vi "sinewave_recovery_array__1dabf32195.vi"(7 "stop steps":i32, 8 "# periods":dbl, 9 "recovery phase (32 points half period)":dbl, 10 "amplitude":dbl=1.0 format="%0.2p", 11 "frequency":dbl=10.0 format="%0.2p") -> (0 "expected duration":dbl, 1 "total points":i32, 2 "Waveform Graph":dbl[](graph), 3 "shear points":dbl)   [LabVIEW 2023]
uses:
  <vilib>/Analysis/NI_AALBase.lvlib
panel:
  out "element":dbl
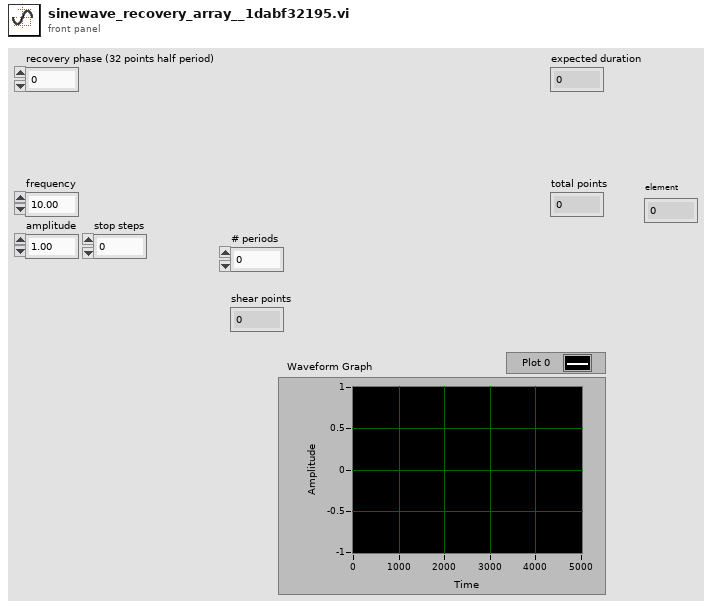
[diagram p1: front panel]
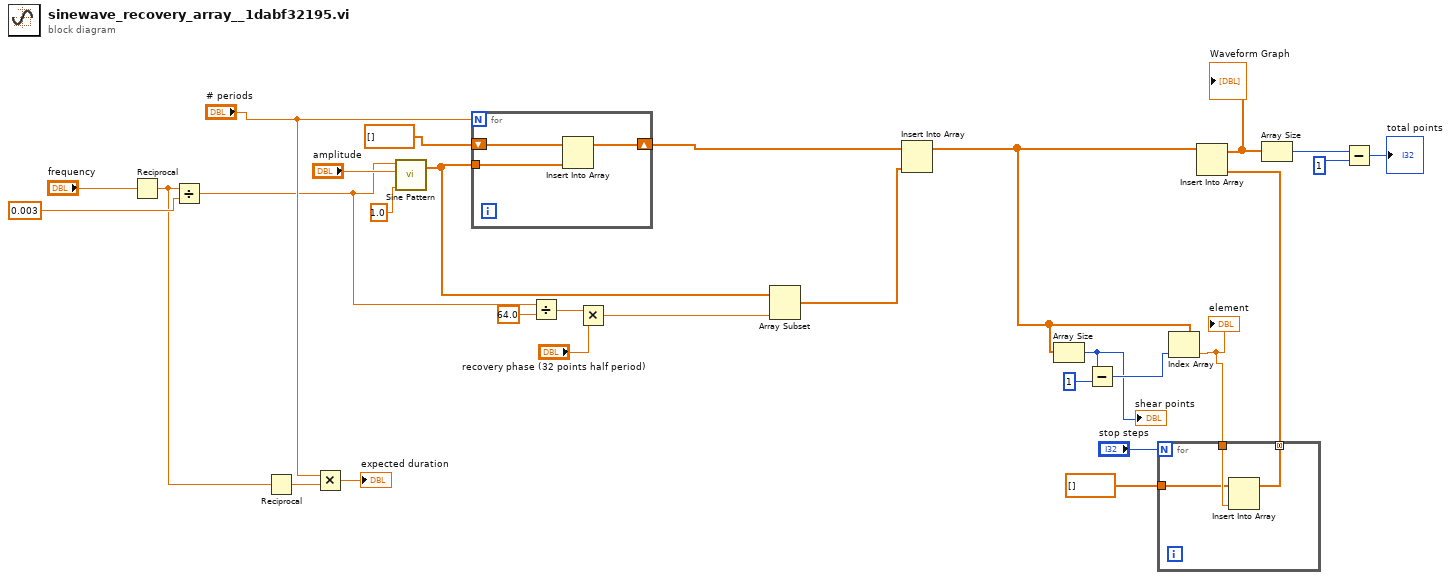
[diagram p0: block diagram]
diagram:
  n1 = Reciprocal(x="frequency") -> (1/x=w1:dbl)
  n2 = Divide(x=w1, y=0.003) -> (x/y=w13:dbl)
  n3 = Reciprocal(x=w1) -> (1/x=w16:dbl)
  n4 = Multiply(x="# periods", y=w16) -> (x*y=→"expected duration":dbl)
  n5 = call <vilib>:"Sine Pattern.vi"("cycles"=1.0, "amplitude"="amplitude", "samples"=w13) -> ("Sinusoidal Pattern"=w8:dbl[])  [unwired: 1 in, 1 out]
  n6 = for {
    N: "# periods" -> [_]
    tunnel: w8 -> [w32]
    shift-right: [w30] -> w5
    shift-left: dbl[] [] ("array") -> [w31]
    n7 = Insert Into Array(array=w31, new element=w32) -> (w30:dbl[])  [unwired: 1 in]
  }
  n8 = Divide(x=w13, y=64.0) -> (x/y=w10:dbl)
  n9 = Multiply(x=w10, y="recovery phase (32 points half period)") -> (x*y=w7:dbl)
  n10 = Array Subset(array=w8, length=w7) -> (w6:dbl[])  [unwired: 1 in]
  n11 = Insert Into Array(array=w5, new element=w6) -> (w4:dbl[])  [unwired: 1 in]
  n12 = Array Size(array=w4) -> (size(s)=w23:i32)
  "shear points" <- w23
  n13 = Subtract(x=w23, y=1) -> (x-y=w28:i32)
  n14 = Index Array(array=w4, index=w28) -> (element=w26:dbl)
  "element" <- w26
  n15 = for {
    N: "stop steps" -> [_]
    tunnel: w26 -> [w35]
    tunnel: [w34] -> w24 mode=concatenating
    tunnel: dbl[] [] ("array") -> [w33]
    n16 = Insert Into Array(array=w33, new element=w35) -> (w34:dbl[])  [unwired: 1 in]
  }
  n17 = Insert Into Array(array=w4, new element=w24) -> (w19:dbl[])  [unwired: 1 in]
  "Waveform Graph" <- w19
  n18 = Array Size(array=w19) -> (size(s)=w18:i32)
  n19 = Subtract(x=w18, y=1) -> (x-y=→"total points":i32)
